vi "Schedule Step.vi"(10 "now":i32, 11 "step":i32) -> (3 "due":i32)   [LabVIEW 2020, in "Full Featured MCP Server.lvlib"]
doc: "Returns the second at which a story step is published: now plus a random delay between delay min and delay max of that step."
uses:
  Full Featured MCP Server.lvlib
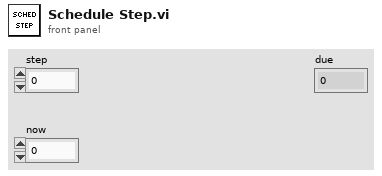
[diagram p1: front panel]
types:
  T1 = cluster{"event":cluster{"headline":string, "scope":enum16{"one stock", "two stocks", "sector", "market"}, "direction":string, "jump":dbl, "follow":dbl, "jump other":dbl, "follow other":dbl}, "delay min":i32, "delay max":i32, "odds":dbl, "next if good":i32, "next if bad":i32}[]
  T2 = cluster{"event":cluster{"headline":string, "scope":enum16{"one stock", "two stocks", "sector", "market"}, "direction":string, "jump":dbl, "follow":dbl, "jump other":dbl, "follow other":dbl}, "delay min":i32, "delay max":i32, "odds":dbl, "next if good":i32, "next if bad":i32}
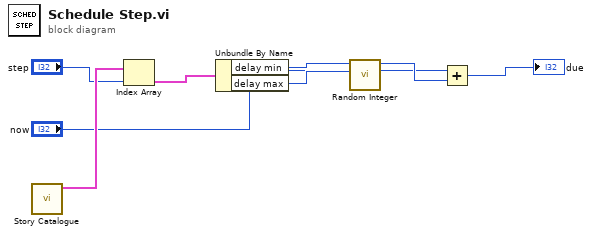
[diagram p0: block diagram]
diagram:
  n1 = call "Story Catalogue.vi"() -> ("steps"=w3:T1)  [unwired: 10 in, 1 out]
  n2 = Index Array(array=w3, index="step") -> (element=w4:T2)
  n3 = Unbundle By Name(w4) -> ("delay min"=w5:i32, "delay max"=w6:i32)
  n4 = call "Random Integer.vi"("high"=w6, "low"=w5) -> ("number"=w7:i32)  [unwired: 9 in]
  n5 = Add(x="now", y=w7) -> (x+y=→"due":i32)
